vi "lvmcp_framediags.vi"() -> ()   [LabVIEW 2026]
panel:
  out "Diagrams[]":refnum<vi>[](array[refnum])
  out "error out":errorcluster
  in  "reference":refnum<vi>
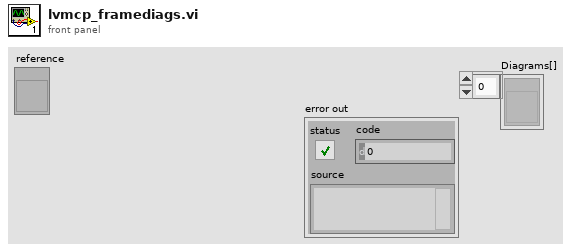
[diagram p1: front panel]
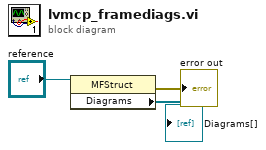
[diagram p0: block diagram]
diagram:
  n1 = property class="MFStruct"(reference="reference") -> (error out=→"error out":errorcluster, "Diagrams"=→"Diagrams[]":refnum<vi>[])  [unwired: 1 in, 1 out]
